vi "Object data correction and extraction.vi"(5 "Object-data-array":dbl[][](array[numeric]), 7 "Object number of interest":i32) -> (0 "Corrected Object orientation":dbl, 1 "Object CoM X":dbl, 2 "Object CoM Y":dbl, 3 "Obejct length":dbl, 4 "Assignment Coordinates":string)   [LabVIEW 2022 SP3]
doc: "Takes the object data array and a insect number and output the coordinates, length and orientation of the chosen object"
panel:
  out "Angle in Range":bool
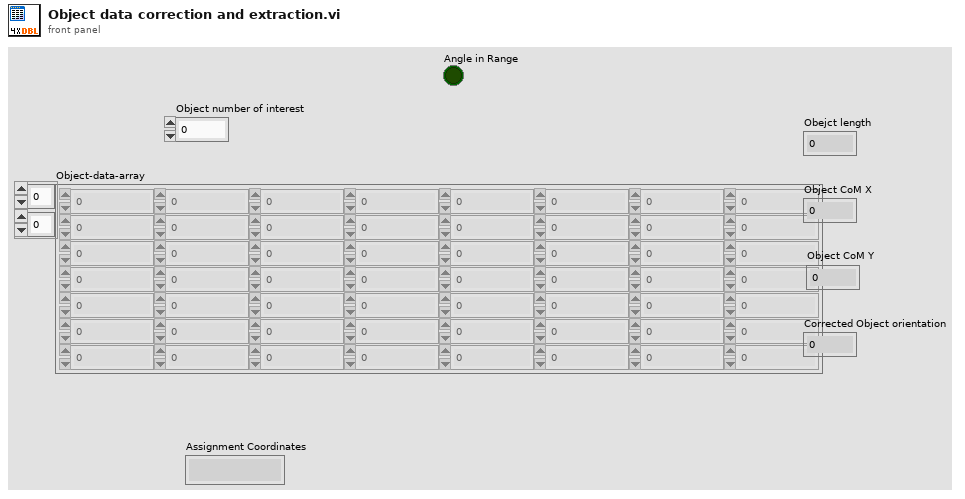
[diagram p1: front panel]
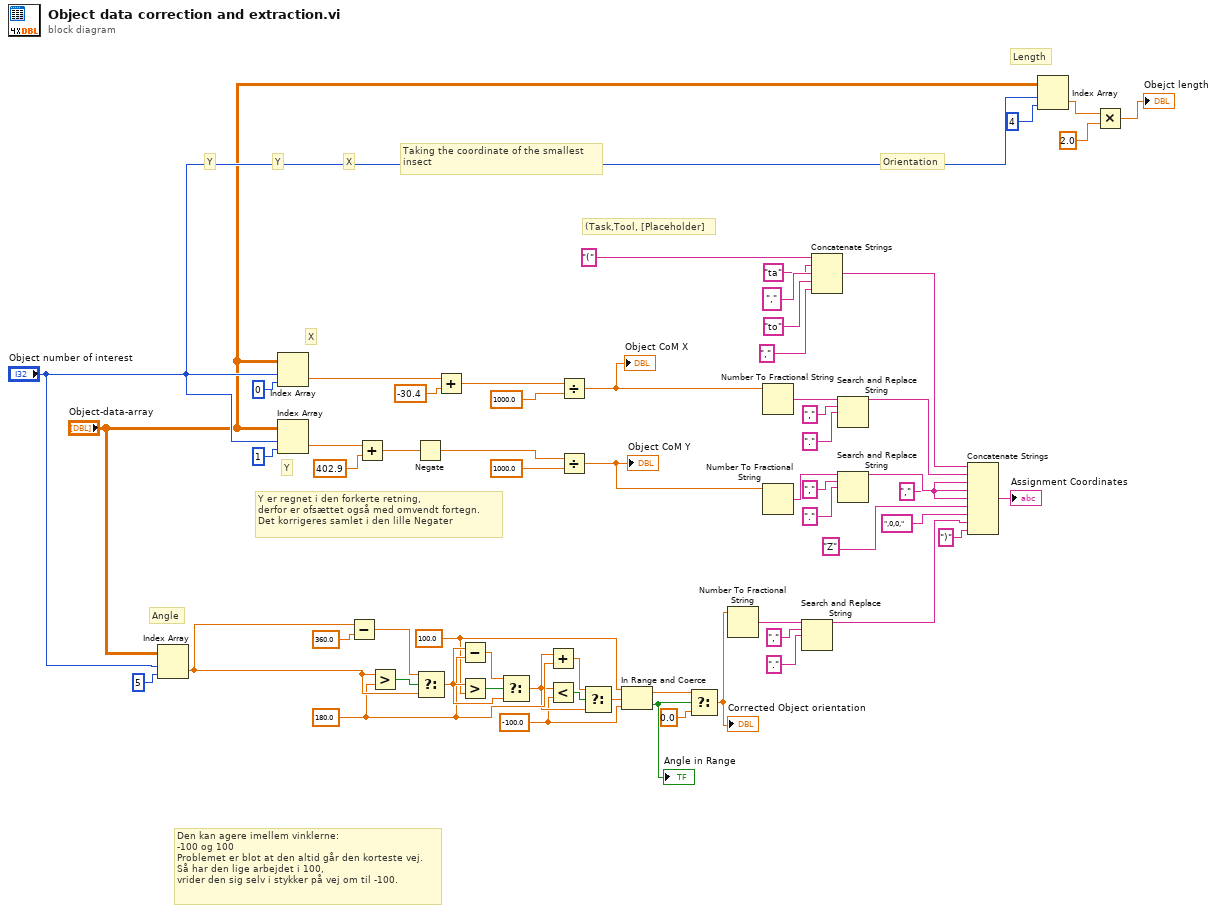
[diagram p0: block diagram]
diagram:
  w5 = -100.0 ("y")
  w9 = 180.0 ("y")
  w6 = 100.0 ("y")
  w26 = "," ("string")
  # "Den kan agere imellem vinklerne:\n-100 og 100\nProblemet er blot at den altid går den korteste vej.\nSå har den lige arbejdet i 100, \nvrider den sig selv i stykker på vej om til -100."
  # "Y er regnet i den forkerte retning, \nderfor er ofsættet også med omvendt fortegn.\nDet korrigeres samlet i den lille Negater"
  # "(Task,Tool, [Placeholder]"
  # "Angle"
  # "Y"
  # "X"
  # "Length"
  # "Taking the coordinate of the smallest \ninsect"
  # "Y"
  # "Orientation"
  # "Y"
  # "X"
  n1 = Index Array(array="Object-data-array", index (row)="Object number of interest", index (col)=5 ("disabled index (col)")) -> (element=w12:dbl)
  n2 = Index Array(array="Object-data-array", index (row)="Object number of interest", index (col)=0 ("disabled index (col)")) -> (element=w50:dbl)
  n3 = Index Array(array="Object-data-array", index (row)="Object number of interest", index (col)=1 ("disabled index (col)")) -> (element=w48:dbl)
  n4 = Subtract(x=w12, y=360.0) -> (x-y=w15:dbl)
  n5 = Add(x=w48, y=402.9) -> (x+y=w51:dbl)
  n6 = Greater?(x=w12, y=w9) -> (0:w16:bool)
  n7 = Negate(x=w51) -> (-x=w54:dbl)
  n8 = Select(t=w15, s=w16, f=w12) -> (s? t:f=w13:dbl)
  n9 = Add(x=w50, y=-30.4) -> (x+y=w55:dbl)
  n10 = Subtract(x=w13, y=w9) -> (x-y=w17:dbl)
  n11 = Greater?(x=w13, y=w6) -> (0:w18:bool)
  n12 = Select(t=w17, s=w18, f=w13) -> (s? t:f=w7:dbl)
  n13 = Add(x=w7, y=w9) -> (x+y=w8:dbl)
  n14 = Less?(x=w7, y=w5) -> (x < y?=w10:bool)
  n15 = Divide(x=w55, y=1000.0) -> (x/y=w28:dbl)
  "Object CoM X" <- w28
  n16 = Divide(x=w54, y=1000.0) -> (x/y=w27:dbl)
  "Object CoM Y" <- w27
  n17 = Select(t=w8, s=w10, f=w7) -> (s? t:f=w11:dbl)
  n18 = In Range and Coerce(upper limit=w6, x=w11, lower limit=w5) -> (coerced(x)=w3:dbl, In Range?=w4:bool)
  "Angle in Range" <- w4
  n19 = Select(t=w3, s=w4, f=0.0) -> (s? t:f=w2:dbl)
  "Corrected Object orientation" <- w2
  n20 = Number To Fractional String(number=w2) -> (F-format string=w36:string)  [unwired: 3 in]
  n21 = Number To Fractional String(number=w28) -> (F-format string=w35:string)  [unwired: 3 in]
  n22 = Number To Fractional String(number=w27) -> (F-format string=w40:string)  [unwired: 3 in]
  n23 = Search and Replace String(input string=w36, search string=",", replace string="." ("replace string (\"\")")) -> (result string=w24:string)  [unwired: 5 in, 3 out]
  n24 = Concatenate Strings("(" ("string"), "ta" ("string"), "," ("string"), "to" ("string"), "," ("string")) -> (w31:string)
  n25 = Search and Replace String(input string=w35, search string=",", replace string="." ("replace string (\"\")")) -> (result string=w43:string)  [unwired: 5 in, 3 out]
  n26 = Search and Replace String(input string=w40, search string=",", replace string="." ("replace string (\"\")")) -> (result string=w39:string)  [unwired: 5 in, 3 out]
  n27 = Concatenate Strings(w31, w43, w26, w39, w26, "Z" ("string"), ",0,0," ("string"), w24, ")" ("string")) -> (→"Assignment Coordinates":string)
  n28 = Index Array(array="Object-data-array", index (row)="Object number of interest", index (col)=4 ("disabled index (col)")) -> (element=w21:dbl)
  n29 = Multiply(x=w21, y=2.0) -> (x*y=→"Obejct length":dbl)
